vi "Create All Message Queues.vi"(8 "error in (no error)":errorcluster) -> (0 "error out":errorcluster, 3 "Message Queues out":T1)   [LabVIEW 2020, in "Message Queue.lvlib"]
doc: "This VI creates and initializes all the message queues for your application. If your application requires more than one message queue, right-click the \"Message Queues\" constant above and select Open Type Def. Add the new Message Queue(s) to the type definition, then initialize them in this VI."
uses:
  Message Queue.lvlib
  Message Cluster.ctl
  All Message Queues.ctl
  adcf10b1-5dc6-4ed0-8602-b119694bc531.vi
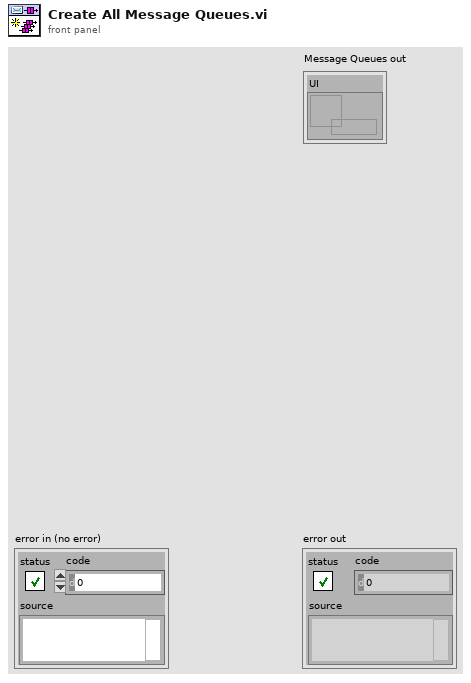
[diagram p1: front panel]
types:
  T1 = typedef "Message Queue.lvlib/All Message Queues.ctl" = cluster{"UI":refnum<queue>}
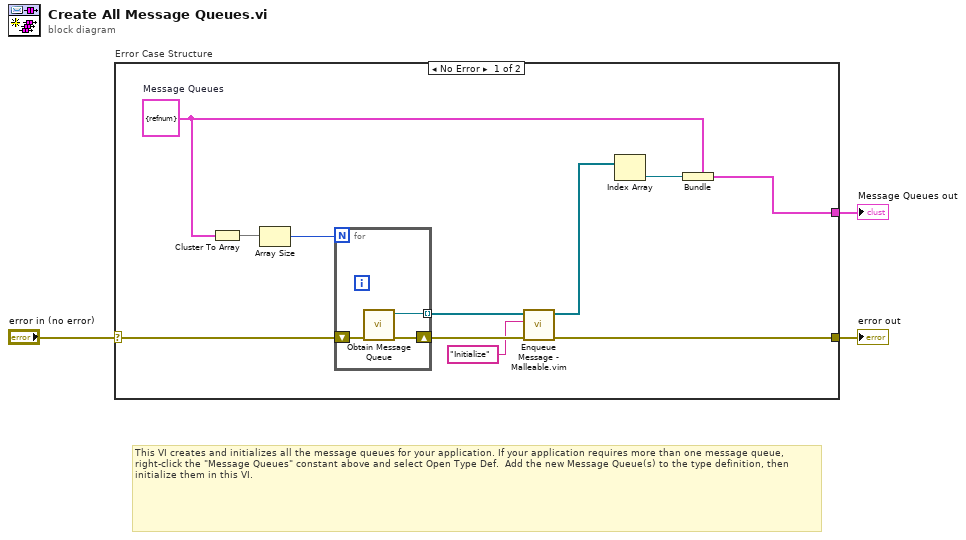
[diagram p0: block diagram]
diagram:
  # "This VI creates and initializes all the message queues for your application. If your application requires more than one message queue, right-click the \"Message Queues\" constant above and select Open Type Def.  Add the new Message Queue(s) to the type definition, then initialize them in this VI."
  n1 = case "Error Case Structure" shown="No Error" "error in (no error)" {
    selector: "error in (no error)" -> [w11 w18]
    tunnel: [w5 w18] -> w3
    tunnel: [w12 _] -> w2
    frame No Error {
      w10 = T1 {"UI"=refnum}  # Message Queues
      n2 = Cluster To Array(cluster=w10) -> (array=w14:refnum<queue>[])
      n3 = Array Size(array=w14) -> (size(s)=w13:i32)
      n4 = for {
        N: w13 -> [_]
        shift-right: [w16] -> w6
        shift-left: w11 -> [w17]
        tunnel: [w15] -> w8 mode=indexing
        n5 = call "Obtain Message Queue.vi"("error in (no error)"=w17) -> ("error out"=w16:errorcluster, "Message Queue"=w15:refnum<queue>)  [unwired: 9 in]
      }
      n6 = call "Enqueue Message - Malleable.vim"("error in (no error)"=w6, "Message"="Initialize", "Message Queue"=w8) -> ("error out"=w5:errorcluster, "dup Message Queue"=w7:refnum<queue>[])  [unwired: 7 in]
      n7 = Index Array "Index Array"(array=w7) -> (element=w9:refnum<queue>)  [unwired: 1 in]
      n8 = Bundle "Bundle"(cluster=w10, "UI"=w9) -> (w12:T1)
    }
    frame Error {
    }
  }
  "Message Queues out" <- w2
  "error out" <- w3
